vi "[ce low] Eval y=f(x1,x2).vi"(0 "Start":cluster{"x1":dbl, "x2":dbl} {"x2" format="%.2f"; "x1" format="%.2f"}, 1 "VC Handle":T2=-1, 2 "number of points":u32=100, 5 "End":cluster{"x1":dbl, "x2":dbl}={"x1"=1.0, "x2"=1.0} {"x2" format="%.2f"; "x1" format="%.2f"}, 7 "offset":cluster{"x1":dbl, "x2":dbl} {"x2" format="%.5e"; "x1" format="%.5e"}, 9 "formula info":T3={"formula"="", "variable 1"="x1", "variable 2"="x2"}, 11 "error in":errorcluster, 12 "vm cmd":T1(ring), 13 "include end point":bool) -> (4 "X1 Values":dbl[](array[numeric]) format="%.2f", 6 "X2  Values":dbl[](array[numeric]) format="%.2f", 8 "Y Values":dbl[][](array[numeric]) format="%.2f", 15 "error out":errorcluster)   [LabVIEW 2021]
doc: "Calculates a 2D array of function values defined on a grid.\n\n::: CalcExpress Toolkit :::\nCopyright (c) 2000-2026 Konstantin Shifershteyn. All rights reserved."
uses:
  cetypes.llb/VarMan Variable Context Handle.ctl
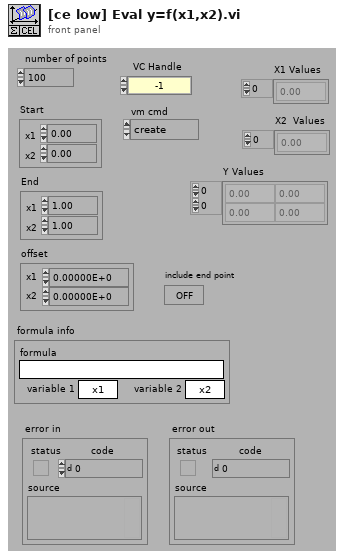
[diagram p1: front panel]
types:
  T1 = enum16{"create", "destroy", "set value", "get value"}
  T2 = typedef "VarMan Variable Context Handle.ctl" = i32
  T3 = cluster{"formula":string, "variable 1":string, "variable 2":string}
  T4 = typedef "CalcExpress Data Type.ctl" = enum32{"String", "DBL Number", "identifier", "1D Array of DBL", "2D Array of DBL", "CDB Number", "1D Array of CDB", "2D Array of CDB", "1D Array of String", "2D Array of String", "Unknown data type"}
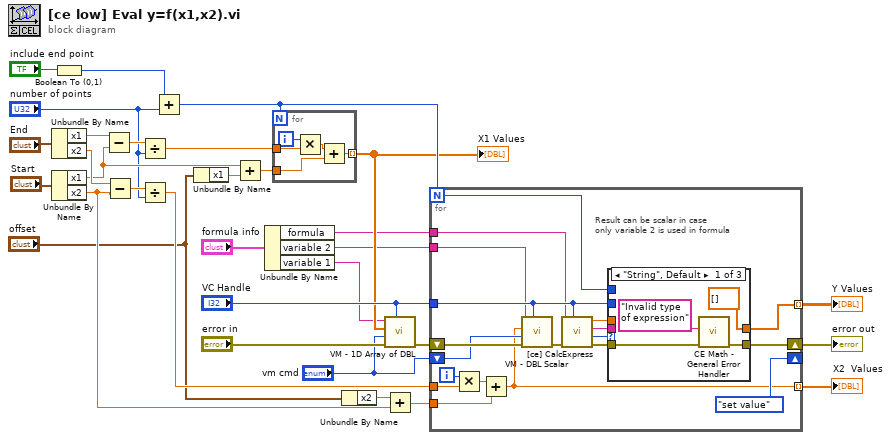
[diagram p0: block diagram]
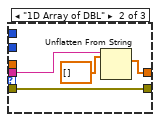
[diagram p2: hidden frame]
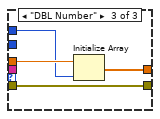
[diagram p3: hidden frame]
diagram:
  n1 = Unbundle By Name("End") -> ("x1"=w26:dbl, "x2"=w29:dbl)
  n2 = Unbundle By Name("Start") -> ("x1"=w15:dbl, "x2"=w14:dbl)
  n3 = Boolean To (0,1)(Boolean="include end point") -> (0, 1=w7:i16)
  n4 = Subtract(x=w26, y=w15) -> (x-y=w28:dbl)
  n5 = Subtract(x=w29, y=w14) -> (x-y=w27:dbl)
  n6 = Divide(x=w28, y="number of points") -> (x/y=w25:dbl)
  n7 = Divide(x=w27, y="number of points") -> (x/y=w19:dbl)
  n8 = Add(x=w7, y="number of points") -> (x+y=w5:u32)
  n9 = Unbundle By Name("offset") -> ("x1"=w10:dbl)
  n10 = Add(x=w15, y=w10) -> (x+y=w11:dbl)
  n11 = Unbundle By Name("formula info") -> ("formula"=w3:string, "variable 2"=w1:string, "variable 1"=w2:string)
  n12 = for {
    N: w5 -> [_]
    tunnel: w25 -> [w33]
    tunnel: [w36] -> w4 mode=indexing
    tunnel: w11 -> [w34]
    i -> [w32]
    n13 = Multiply(x=w32, y=w33) -> (x*y=w35:dbl)
    n14 = Add(x=w35, y=w34) -> (x+y=w36:dbl)
  }
  "X1 Values" <- w4
  n15 = Unbundle By Name("offset") -> ("x2"=w12:dbl)
  n16 = call "VM - 1D Array of DBL.vi"("VC Handle"="VC Handle", "error in"="error in", "cmd"="vm cmd", "value in"=w4, "name_spec"=w2) -> ("error out"=w21:errorcluster)  [unwired: 1 in, 5 out]
  n17 = Add(x=w12, y=w14) -> (x+y=w13:dbl)
  n18 = for {
    N: w5 -> [w37]
    tunnel: "VC Handle" -> [w54]
    tunnel: [w53] -> w17 mode=indexing
    tunnel: w1 -> [w52]
    tunnel: w3 -> [w51]
    shift-right: [w49] -> w18
    shift-left: w21 -> [w48]
    shift-right: [T1."set value" ("vm cmd")] -> _
    shift-left: "vm cmd" -> [w47]
    tunnel: w19 -> [w43]
    tunnel: w13 -> [w42]
    tunnel: [w41] -> w16 mode=indexing
    i -> [w45]
    # "Result can be scalar in case\nonly variable 2 is used in formula"
    n19 = Multiply(x=w45, y=w43) -> (x*y=w44:dbl)
    n20 = Add(x=w44, y=w42) -> (x+y=w41:dbl)
    n21 = call "VM - DBL Scalar.vi"("VC Handle"=w54, "error in"=w48, "cmd"=w47, "value in"=w41, "name_spec"=w52) -> ("error out"=w50:errorcluster)  [unwired: 1 in, 5 out]
    n22 = call "[ce] CalcExpress.vi"("VC Handle"=w54, "error in"=w50, "expression"=w51) -> ("error out"=w55:errorcluster, "value type"=w40:T4, "string value"=w38:string, "numeric value"=w39:dbl)  [unwired: 3 in]
    n23 = case shown="\"String\", Default" w40 {
      tunnel: w55 -> [w58 w63 w67]
      tunnel: w54 -> [_ _ _]
      tunnel: [dbl[] [] ("value out") w62 w65] -> w53
      tunnel: [w57 w63 w67] -> w49
      tunnel: w39 -> [_ _ w66]
      tunnel: w37 -> [_ _ w64]
      tunnel: w38 -> [_ w61 _]
      frame "String", Default {
        n24 = call "CE Math - General Error Handler.vi"("error before"=w58, "message"="Invalid type of expression") -> ("error out"=w57:errorcluster)  [unwired: 6 in, 1 out]
      }
      frame "1D Array of DBL" {
        n25 = Unflatten From String(type=dbl[] [] ("X1 Values"), binary string=w61) -> (value=w62:dbl[])  [unwired: 3 in, 2 out]
      }
      frame "DBL Number" {
        n26 = Initialize Array(w66, w64) -> (w65:dbl[])
      }
    }
  }
  "Y Values" <- w17
  "X2  Values" <- w16
  "error out" <- w18
